vi "BB Raw Reader from Refnum.vi"(3 "BB Raw Reader Refnum":T1 {"refnum" format="%.0x"}) -> (5 "BB Raw Reader U64":u64)   [LabVIEW 2021, in "Iceoryx.lvlib"]
uses:
  Iceoryx.lvlib
  Typedef/BB Raw Reader Refnum.ctl
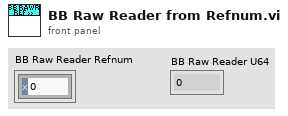
[diagram p1: front panel]
types:
  T1 = typedef "Iceoryx.lvlib/BB Raw Reader Refnum.ctl" = cluster{"refnum":u64, "BB Raw Reader":enum8{"bb_raw_reader"}}
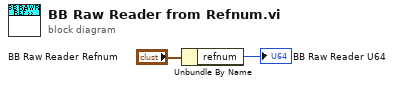
[diagram p0: block diagram]
diagram:
  n1 = Unbundle By Name("BB Raw Reader Refnum") -> ("refnum"=→"BB Raw Reader U64":u64)
